vi "gdi32 GetDIBits.vi"(0 "hdc":u64, 1 "hbm":u64, 2 "start":u32, 3 "cLines":u32, 4 "lpvBits":u32[](array[numeric]), 5 "lpbmi":T1={"biSize"=40, "biWidth"=0, "biHeight"=0, "biPlanes"=1, "biBitCount"=32, "biCompression"=0, "biSizeImage"=0, "biXPelsPerMeter"=0, "biYPelsPerMeter"=0, "biClrUsed"=0, "biClrImportant"=0, "bmiColors"=0}, 6 "usage":u32, 7 "error in":errorcluster) -> (20 "lpvBits out":u32[](array[numeric]), 21 "return value":i32, 27 "error out":errorcluster)   [LabVIEW 2020, in "RemoteVI.lvlib"]
doc: "Copies scan lines of the bitmap hbm into lpvBits in the format lpbmi describes, through gdi32.dll GetDIBits (stdcall, called in any thread). hbm must NOT be selected into a device context at the time. For 32-bit pixels set lpbmi to biSize 40, biWidth w, biHeight -h (top-down rows), biPlanes 1, biBitCount 32, biCompression 0 (BI_RGB), and preallocate lpvBits with w*h elements; each pixel then reads 0xXXRRGGBB. lpbmi is a BITMAPINFOHEADER plus one spare 32-bit colour entry (44 bytes). return value is the number of lines copied, 0 on failure. When error in carries an error the DLL is not called. Generated by scripts\\Build Win32 Wrappers.vi - do not edit by hand, rebuild it."
uses:
  RemoteVI.lvlib
  gdi32.dll
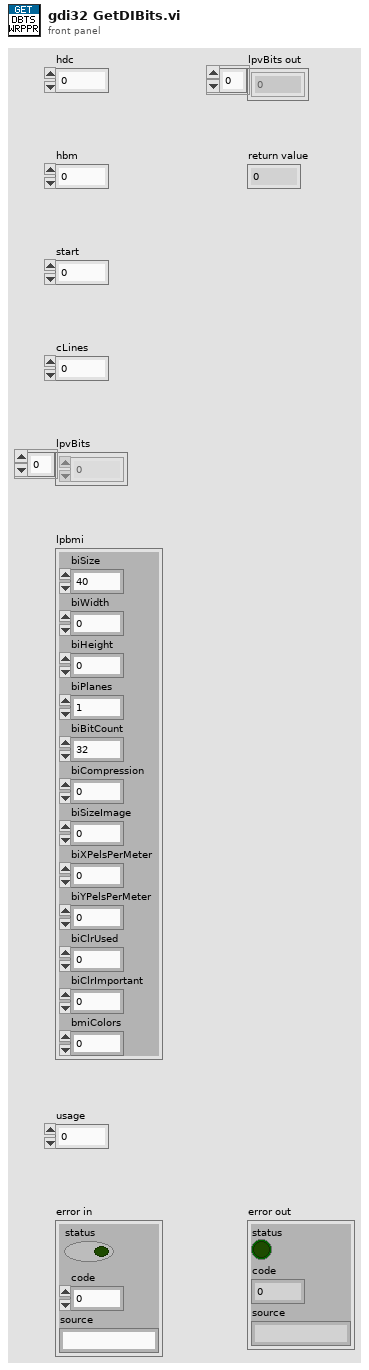
[diagram p1: front panel]
types:
  T1 = cluster{"biSize":u32, "biWidth":i32, "biHeight":i32, "biPlanes":u16, "biBitCount":u16, "biCompression":u32, "biSizeImage":u32, "biXPelsPerMeter":i32, "biYPelsPerMeter":i32, "biClrUsed":u32, "biClrImportant":u32, "bmiColors":u32}
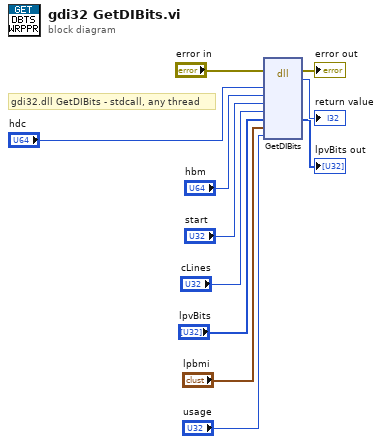
[diagram p0: block diagram]
diagram:
  # "gdi32.dll GetDIBits - stdcall, any thread"
  n1 = dll-call lib="gdi32.dll" fn="GetDIBits"(error in="error in", "hdc"="hdc", "hbm"="hbm", "start"="start", "cLines"="cLines", "lpvBits"="lpvBits", "lpbmi"="lpbmi", "usage"="usage") -> (error out=→"error out":errorcluster, →"return value":i32, "lpvBits"=→"lpvBits out":u32[])  [unwired: 8 in, 1 out]
